vi "Standard Engine.vi"(8 "error in":errorcluster, 9 "status notifier":refnum<notifier>, 10 "rt fifo":refnum<k33>, 11 "Engine Data":T1={"Main Tag Data"={"Double"=[], "Single"=[], "I64"=[], "I32"=[], "I16"=[], "I8"=[], "U64"=[], "U32"=[], "U16"=[], "U8"=[], "Boolean"=[], "String"=[], "Array of Double"=[], "Array of Single"=[], "Array of I64"=[], "Array of I32"=[], "Array of I16"=[], "Array of I8"=[], "Array of U64"=[], "Array of U32"=[], "Array of U16"=[], "Array of U8"=[], "Array of Boolean"=[], "Array of String"=[]}, "Module Info"={"Tag Bus Modules"=[], "Input Method Indices"=[], "Process Method Indices"=[], "Output Method Indices"=[], "Input Transfer Specifications"=[], "Parameter Transfer Specifications"=[], "Result Transfer Specifications"=[], "Output Transfer Specifications"=[], "Module Errors"=[], "UID"=""}, "Safe State?"=FALSE, "engine timing source"=refnum, "Processor"=-2, "Priority"=1, "dT"=0}) -> (0 "error out":errorcluster)   [LabVIEW 2014, in "synchronous engine runtime.lvclass"]
uses:
  synchronous engine runtime.lvclass
  Engine Data.ctl
  <vilib>/NI/Module Timing Source/timing source/TBM timing source.lvclass
  <vilib>/NI/Tag Bus/table/data table.ctl
  Module Execution Info.ctl
  <vilib>/NI/Tag Bus Module Framework/runtime/TBM module execution interface.lvclass
  Data Table with Transfer Spec.ctl
  <vilib>/NI/Tag Bus/table/transfer specification.ctl
  <vilib>/NI/Tag Bus/tag/Data Type.ctl
  Commands.ctl
  notifier.ctl
  Engine Runtime/Execution States.ctl
  Engine Runtime/Engine Runtime Interface.lvclass
  <vilib>/Platform/TimedLoop/XDataNode/XDataNode.xnode
  <vilib>/Platform/TimedLoop/XDataNode/nitl_modes.ctl
  <vilib>/Platform/TimedLoop/XDataNode/XDNodeRunTimeDep.lvlib
  <vilib>/Platform/TimedLoop/XDataNode/wakeup.ctl
  <vilib>/Platform/TimedLoop/XDataNode/timing_clust.ctl
  <vilib>/NI/Tag Bus/table/data table.lvlib
  <vilib>/NI/Tag Bus/tag/tag descriptor.lvclass
panel:
  out "iterations":i32
  in  "Network Address":string="10.1.128.117"
  in  "send trace?":bool
  out "loop period (ms)":u32
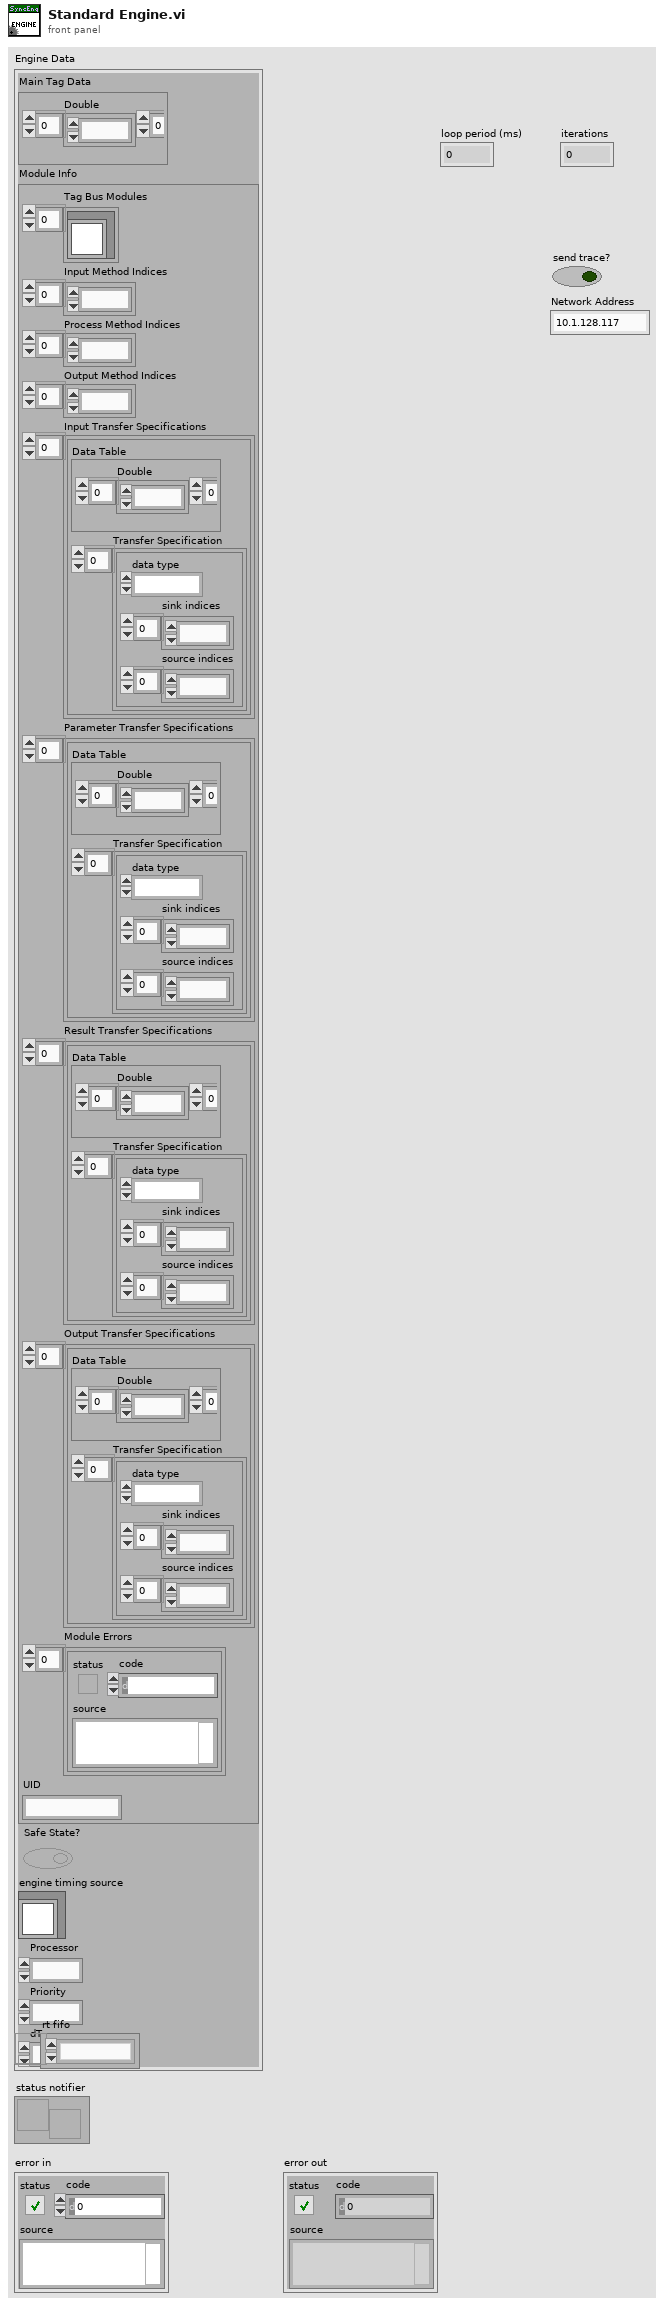
[diagram p1: front panel]
types:
  T1 = typedef "synchronous engine runtime.lvclass/Engine Data.ctl" = cluster{"Main Tag Data":T2, "Module Info":T3, "Safe State?":bool, "engine timing source":refnum<class "TBM timing source.lvclass">, "Processor":i32, "Priority":i32, "dT":u32}
  T2 = typedef "tag bus.lvlib/data table.lvlib/data table.ctl" = cluster{"Double":dbl[], "Single":sgl[], "I64":i64[], "I32":i32[], "I16":i16[], "I8":i8[], "U64":u64[], "U32":u32[], "U16":u16[], "U8":u8[], "Boolean":bool[], "String":string[], "Array of Double":cluster{"DBL Array":dbl[]}[], "Array of Single":cluster{"SGL Array":sgl[]}[], "Array of I64":cluster{"I64 Array":i64[]}[], "Array of I32":cluster{"I32 Array":i32[]}[], "Array of I16":cluster{"I16 Array":i16[]}[], "Array of I8":cluster{"I8 Array":i8[]}[], "Array of U64":cluster{"U64 Array":u64[]}[], "Array of U32":cluster{"U32 Array":u32[]}[], "Array of U16":cluster{"U16 Array":u16[]}[], "Array of U8":cluster{"U8 Array":u8[]}[], "Array of Boolean":cluster{"Boolean Array":bool[]}[], "Array of String":cluster{"String Array":string[]}[]}
  T3 = typedef "synchronous engine runtime.lvclass/Module Execution Info.ctl" = cluster{"Tag Bus Modules":refnum<class "TBM module execution interface.lvclass">[], "Input Method Indices":i32[], "Process Method Indices":i32[], "Output Method Indices":i32[], "Input Transfer Specifications":T4[], "Parameter Transfer Specifications":T4[], "Result Transfer Specifications":T4[], "Output Transfer Specifications":T4[], "Module Errors":errorcluster[], "UID":string}
  T4 = typedef "synchronous engine runtime.lvclass/Data Table with Transfer Spec.ctl" = cluster{"Data Table":T2, "Transfer Specification":T5[]}
  T5 = typedef "tag bus.lvlib/data table.lvlib/transfer specification.ctl" = cluster{"data type":T6, "sink indices":i32[], "source indices":i32[]}
  T6 = typedef "tag bus.lvlib/tag descriptor.lvclass/Data Type.ctl" = enum16{"Double", "Single", "I64", "I32", "I16", "I8", "U64", "U32", "U16", "U8", "Boolean", "String", "Array of Double", "Array of Single", "Array of I64", "Array of I32", "Array of I16", "Array of I8", "Array of U64", "Array of U32", "Array of U16", "Array of U8", "Array of Boolean", "Array of String"}
  T7 = typedef "Engine Runtime Interface.lvclass/Execution States.ctl" = enum16{"Init", "Pre-Operational", "Safe-Operational", "Operational", "Stopped"}
  T8 = typedef "synchronous engine runtime.lvclass/notifier.ctl" = cluster{"Engine State":T7, "error constant":errorcluster}
  T9 = typedef "synchronous engine runtime.lvclass/Commands.ctl" = enum16{"Start", "Pause", "Safe State", "Normal", "Stop", "Shutdown"}
  T10 = typedef "XDNodeRunTimeDep.lvlib/timing_clust.ctl" = cluster{"Expected End [f-1]":u64, "Actual End [f-1]":u64, "Finished Late? [f-1]":bool, "Expected End [i-1]":u64, "Actual End [i-1]":u64, "Finished Late? [i-1]":bool, "Expected Start [i]":u64, "Actual Start [i]":u64, "Expected Start [f]":u64, "Actual Start [f]":u64, "Source Name":string, "Structure Name":string, "Period":i64, "Deadline":i64, "Offset":i64, "Start":i64, "Priority":i32, "Timeout":i32, "Mode":T11, "Wakeup Reason":T12, "Error":errorcluster, "Source Type":string, "Secondary Source Type":string, "Global End Time":u64, "Global Start Time":u64, "Frame Duration":u64, "Iteration Duration":u64, "Assigned CPU":i32, "I/O Scan Engine Mode":u32}
  T11 = typedef "XDNodeRunTimeDep.lvlib/nitl_modes.ctl" = enum32{"No Change", "Process missed periods, maintain original phase", "Discard missed periods, maintain original phase", "Process missed periods, ignore original phase", "Discard missed periods, ignore original phase"}
  T12 = typedef "XDNodeRunTimeDep.lvlib/wakeup.ctl" = enum32{"Normal", "Aborted", "Asynchronous wakeup", "Timing source error", "Timed loop error", "Timeout"}
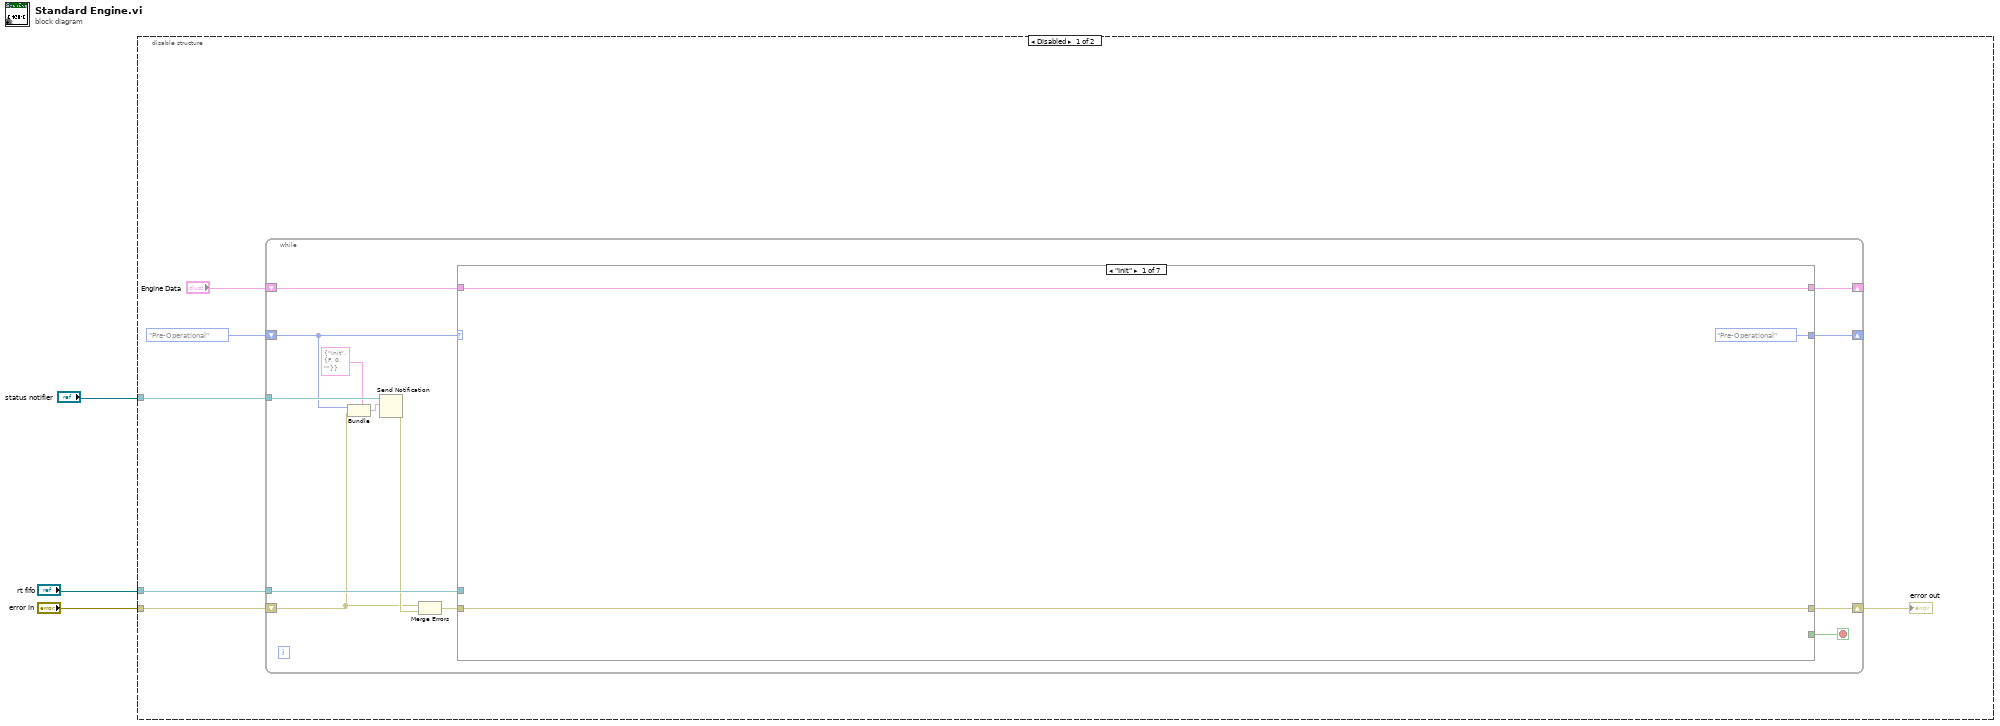
[diagram p0: block diagram]
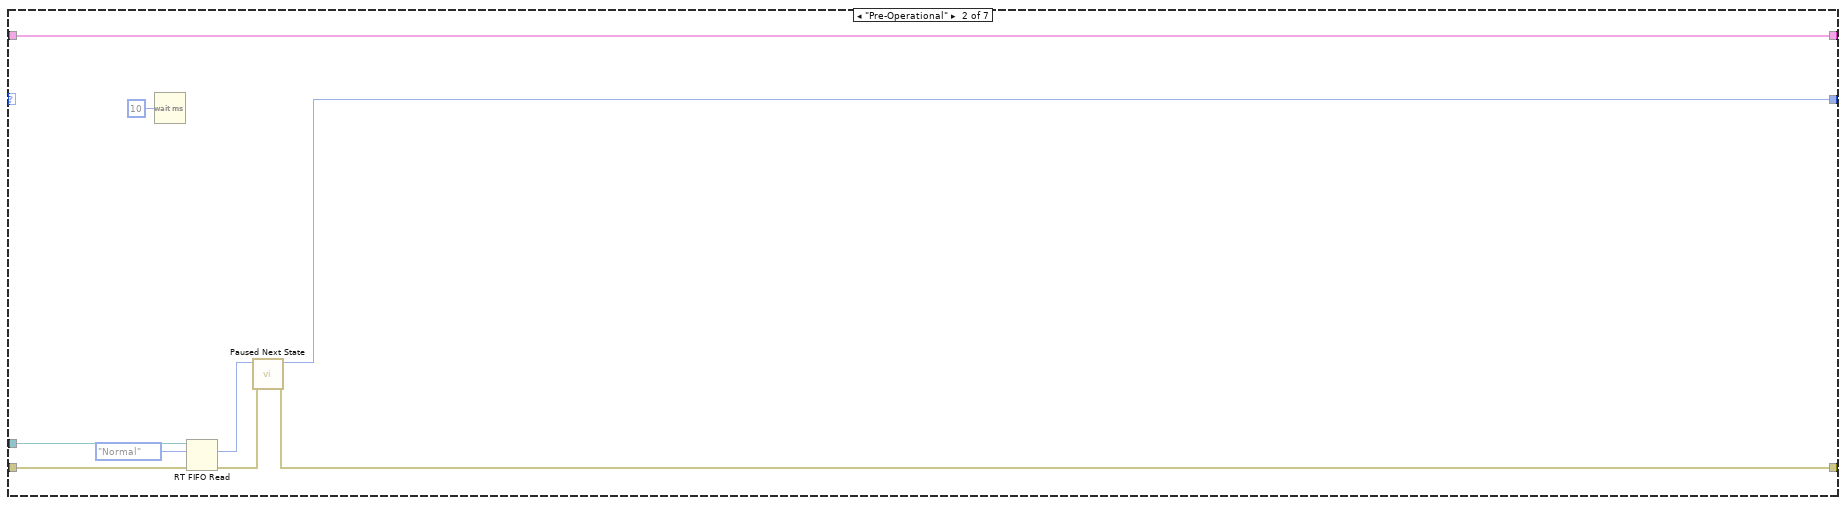
[diagram p2: hidden frame]
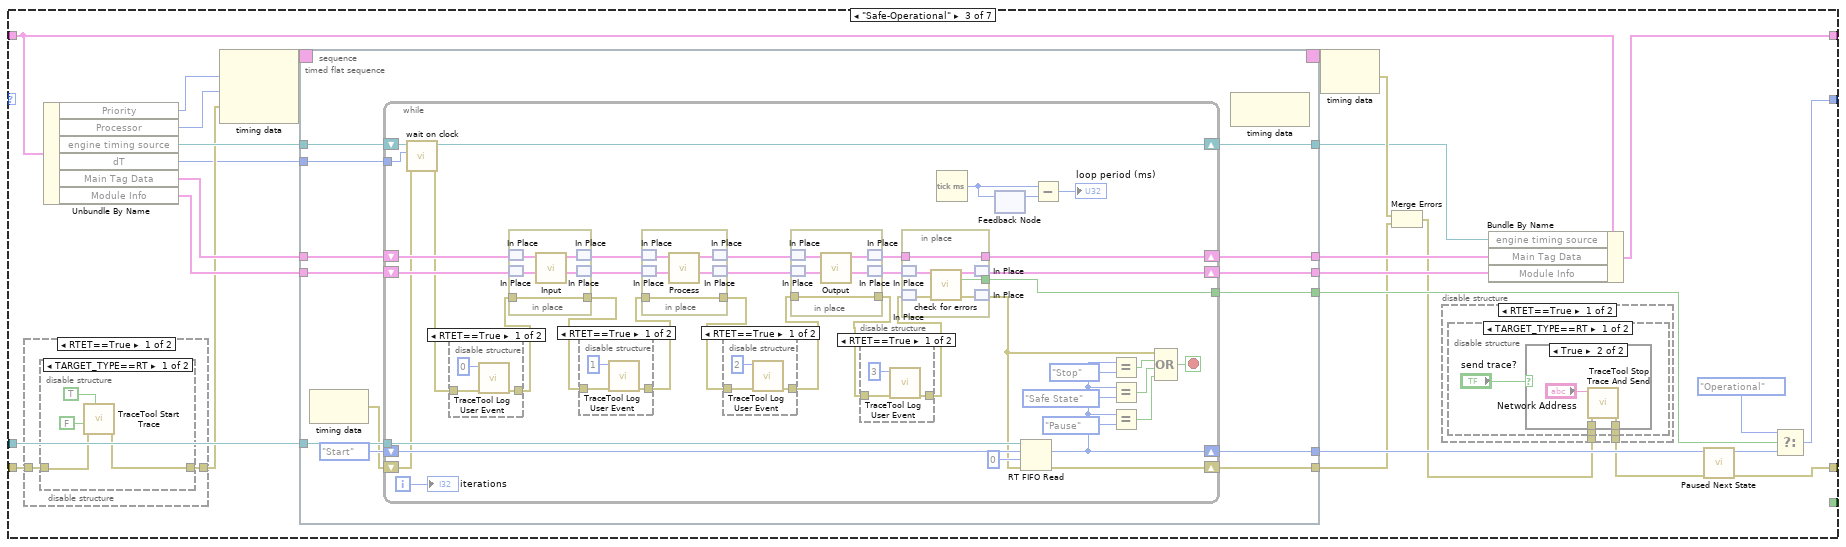
[diagram p3: hidden frame]
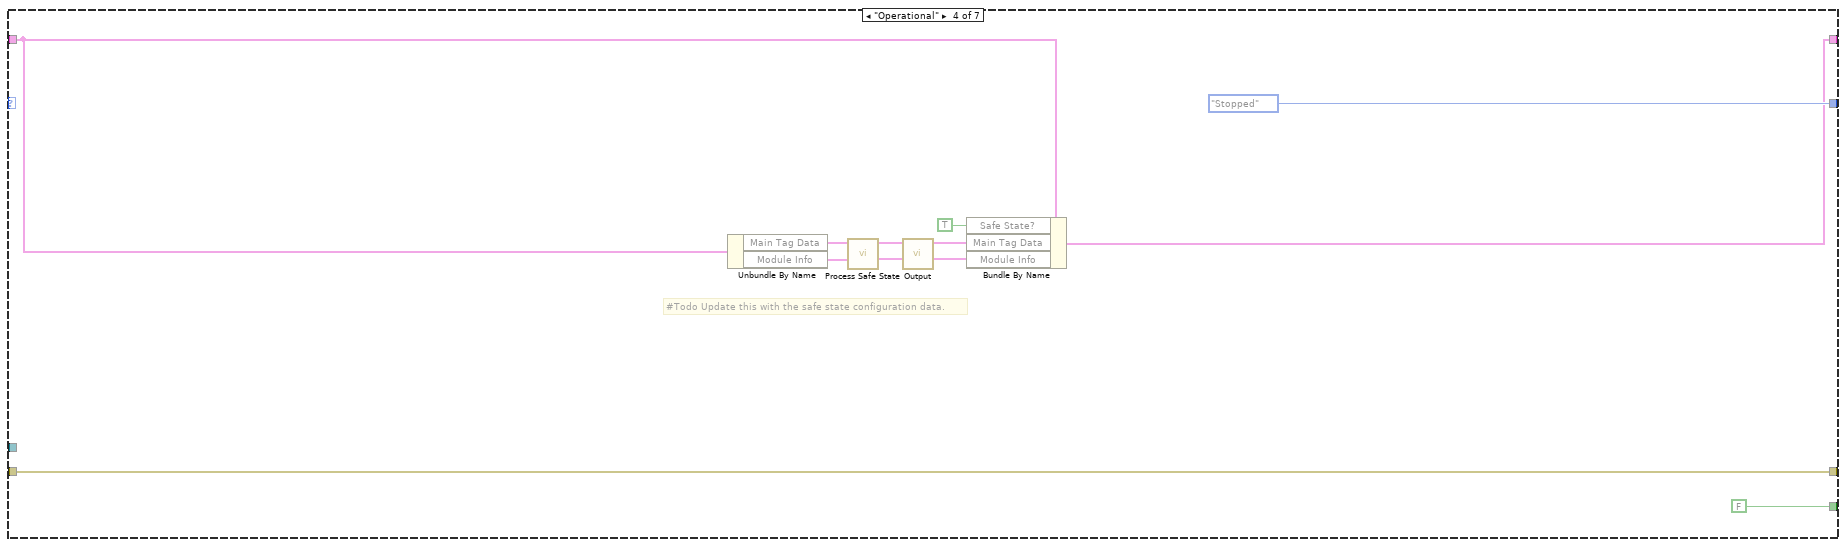
[diagram p13: hidden frame]
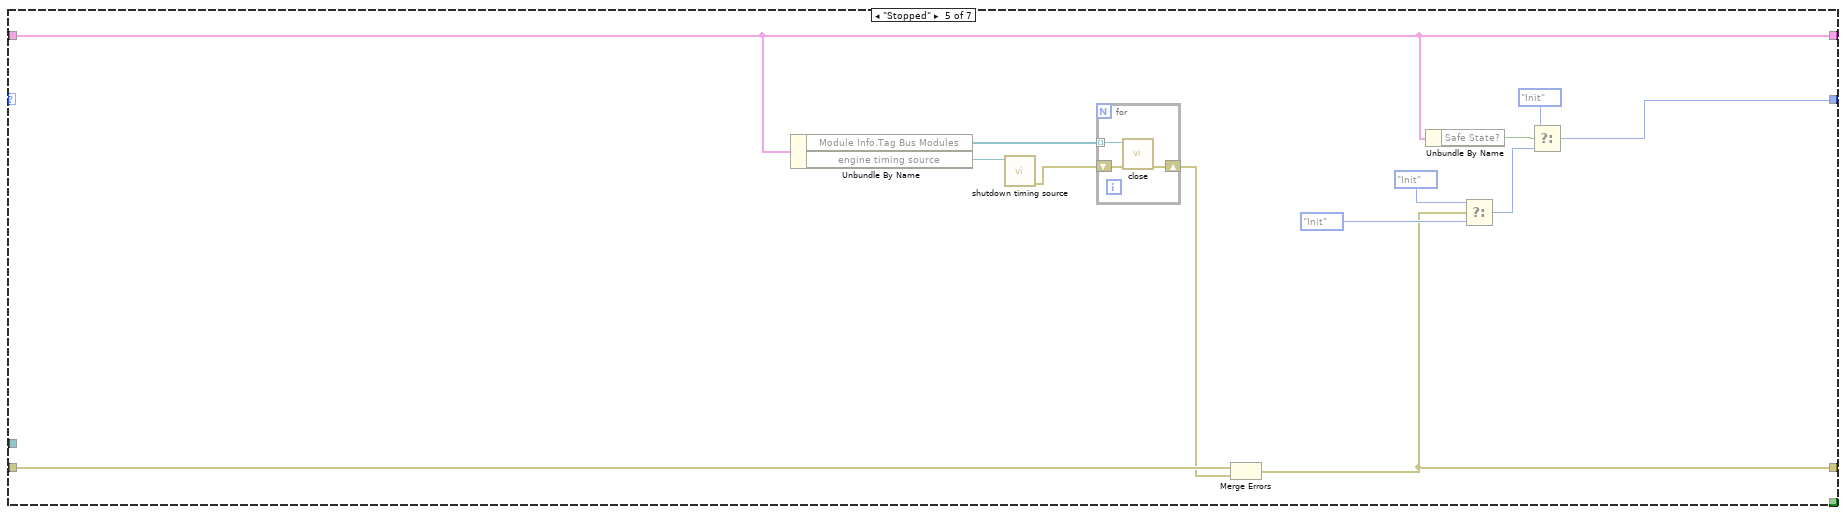
[diagram p14: hidden frame]
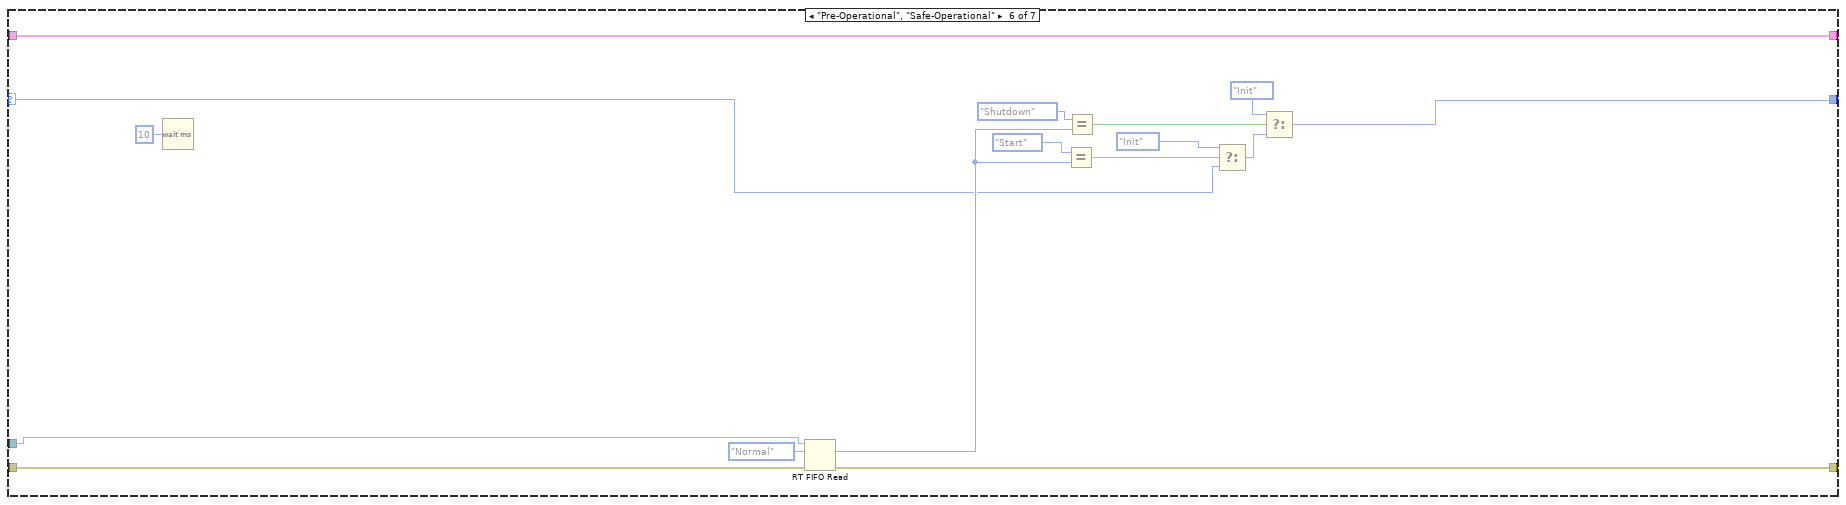
[diagram p15: hidden frame]
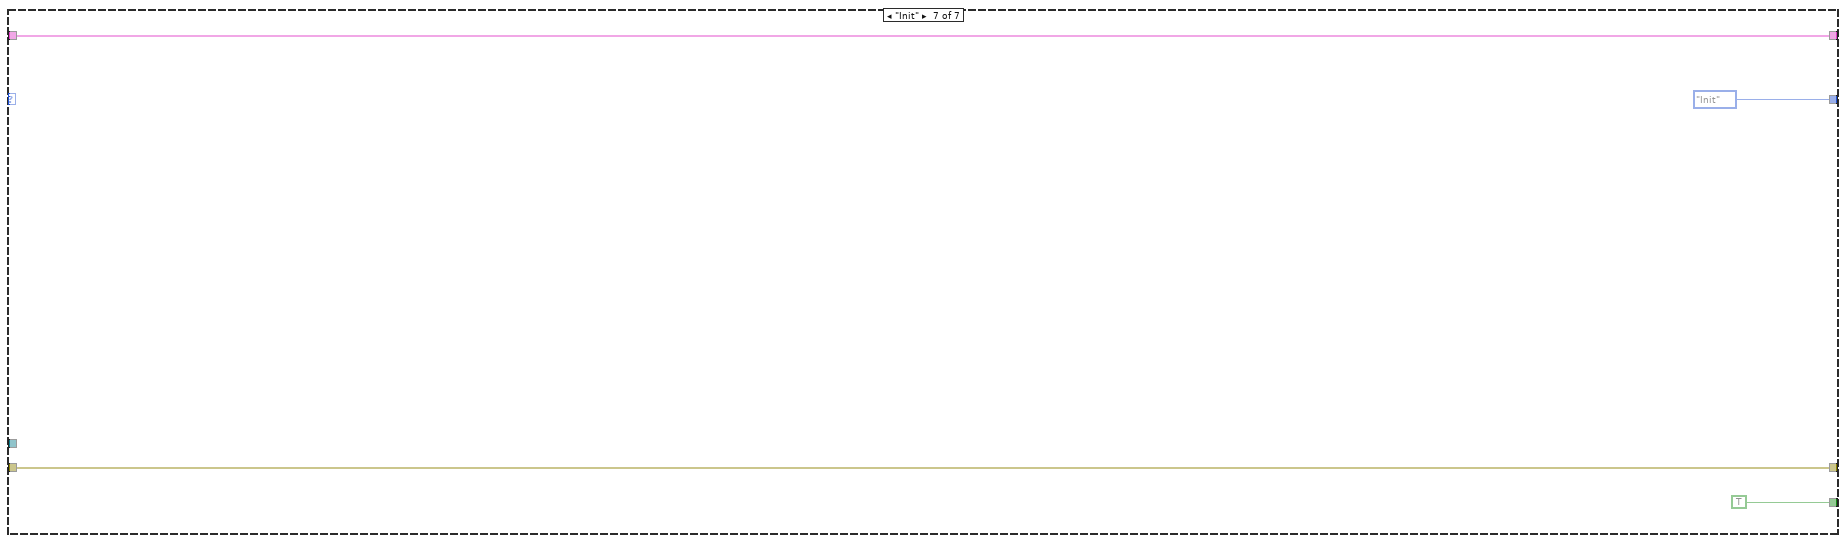
[diagram p16: hidden frame]
diagram:
  n1 = disable-structure shown="Disabled" {
    disable-tunnel: "error in" -> [w7 _]
    disable-tunnel: "status notifier" -> [w6 _]
    disable-tunnel: "rt fifo" -> [w4 _]
    frame Disabled {
      n2 = while {
        shift-right: [w19] -> _
        shift-left: Execution_States."Pre-Operational" ("States") -> [w13]
        shift-right: [w20] -> _
        shift-left: "Engine Data" -> [w22]
        shift-right: [w21] -> w8
        shift-left: w7 -> [w10]
        tunnel: w4 -> [w18]
        tunnel: w6 -> [w16]
        stop <- w17 stop-if-true
        n3 = Bundle(cluster=T8 {"Engine State"=enum."Init", "error constant"={"status"=FALSE, "code"=0, "source"=""}} ("notification"), "Engine State"=w13, "error constant"=w10) -> (w12:T8)
        n4 = Send Notification(notification=w12, notifier=w16) -> (error out=w15:errorcluster)  [unwired: 1 in, 1 out]
        n5 = Merge Errors(w10, w15) -> (w11:errorcluster)
        n6 = case shown="\"Init\"" w13 {
          selector: w13 -> [_ _ _ _ _ w220 _]
          tunnel: w22 -> [w25 w34 w36 w194 w204 w219 w236]
          tunnel: w11 -> [w24 w33 w48 w202 w208 w222 w238]
          tunnel: [w24 w27 w53 w202 w206 w229 w238] -> w21
          tunnel: [w25 w34 w37 w193 w204 w219 w236] -> w20
          tunnel: [Execution_States."Pre-Operational" ("States") w31 w49 Execution_States."Stopped" ("States") w210 w231 Execution_States."Init" ("States")] -> w19
          tunnel: w18 -> [_ w26 w60 _ _ w221 _]
          tunnel: [_ _ _ FALSE _ _ TRUE] -> w17
          frame "Init" {
          }
          frame "Pre-Operational" {
            n7 = Wait (ms)(milliseconds to wait=u32 10) -> ()  [unwired: 1 out]
            n8 = RT FIFO Read(0:w26, 1:Commands."Normal" ("Commands"), 3:w33) -> (9:w30:T9, 11:w29:errorcluster)  [unwired: 1 in, 3 out]
            n9 = call "Paused Next State.vi"("error in"=w29, "Command"=w30) -> ("error out"=w27:errorcluster, "State"=w31:T7)  [unwired: 8 in]
          }
          frame "Safe-Operational" {
            n10 = disable-structure shown="RTET==True" {
              disable-tunnel: w48 -> [w184 w190]
              disable-tunnel: [w183 w190] -> w43
              frame condition #0 {
                n11 = disable-structure shown="TARGET_TYPE==RT" {
                  disable-tunnel: w184 -> [w185 w189]
                  disable-tunnel: [w186 w189] -> w183
                  frame condition #0 {
                    n12 = call <vilib>:"TraceTool Start Trace.vi"("Detailed Tracing? (F)"=TRUE, "error in (no error)"=w185, "VI Tracing? (T)"=FALSE) -> ("error out"=w186:errorcluster)  [unwired: 7 in, 1 out]
                  }
                  frame condition #1 (active) {
                  }
                }
              }
              frame condition #1 (active) {
              }
            }
            n13 = Unbundle By Name(w36) -> ("Priority"=w38:i32, "Processor"=w39:i32, "engine timing source"=w44:refnum<class "TBM timing source.lvclass">, "dT"=w35:u32, "Main Tag Data"=w59:T2, "Module Info"=w58:T3)
            n14 = node-c288(w38, w39, w43) -> (w41:T10)
            n15 = timed-sequence {
              timing: w41 -> [_]
              timing-out: [_] -> w40
              tunnel: w60 -> [w71]
              tunnel: w59 -> [w70]
              tunnel: w58 -> [w69]
              tunnel: [w68] -> w57
              tunnel: [w67] -> w56
              tunnel: [w66] -> w55
              tunnel: [w65] -> w51
              tunnel: [w64] -> w47
              tunnel: w44 -> [w62]
              tunnel: [w63] -> w42
              tunnel: w35 -> [w61]
              n16 = timed-flat-sequence {
                tunnel: w71 -> [w84]
                tunnel: w70 -> [w82]
                tunnel: w69 -> [w81]
                tunnel: [w80] -> w68
                tunnel: [w79] -> w67
                tunnel: [w78] -> w66
                tunnel: [w77] -> w65
                tunnel: [w75] -> w64
                tunnel: [w74] -> w63
                tunnel: w62 -> [w73]
                tunnel: w61 -> [w72]
                n17 = node-c288() -> (w76:errorcluster)  [unwired: 1 in]
                n18 = while {
                  tunnel: w84 -> [w107]
                  shift-right: [w115] -> w78
                  shift-left: Commands."Start" ("Commands") -> [w127]
                  shift-right: [w104] -> w80
                  shift-left: w82 -> [w125]
                  shift-right: [w119] -> w79
                  shift-left: w81 -> [w124]
                  tunnel: [w102] -> w77
                  shift-right: [w106] -> w75
                  shift-left: w76 -> [w91]
                  shift-right: [w89] -> w74
                  shift-left: w73 -> [w92]
                  tunnel: w72 -> [w88]
                  i -> [w101]
                  stop <- w108 stop-if-true
                  n19 = call-dynamic "wait on clock.vi"("error in"=w91, "dt"=w88, "timing source in"=w92) -> ("error out"=w90:errorcluster, "timing source out"=w89:refnum<class "TBM timing source.lvclass">)  [unwired: 6 in, 1 out]
                  n20 = disable-structure shown="RTET==True" {
                    disable-tunnel: w90 -> [w142 w143]
                    disable-tunnel: [w141 w143] -> w99
                    frame condition #0 {
                      n21 = call <vilib>:"TraceTool Log User Event.vi"("error in (no error)"=w142, "Event ID (0-255)"=u32 0) -> ("error out"=w141:errorcluster)  [unwired: 9 in]
                    }
                    frame condition #1 (active) {
                    }
                  }
                  n22 = in-place {
                    in-place-border: w99 -> [w164]
                    in-place-border: [w164] -> w98
                    n23 = in-place-match #1(w125) -> (w163:T2)
                    n24 = in-place-match #2(w124) -> (w160:T3)
                    n25 = call "Input.vi"("Module Info In"=w160, "Engine Tags In"=w163) -> ("Module Info Out"=w161:T3, "Engine Tags Out"=w162:T2)  [unwired: 8 in]
                    n26 = in-place-match #1(w162) -> (w123:T2)
                    n27 = in-place-match #2(w161) -> (w122:T3)
                  }
                  n28 = disable-structure shown="RTET==True" {
                    disable-tunnel: w98 -> [w138 w139]
                    disable-tunnel: [w137 w139] -> w97
                    frame condition #0 {
                      n29 = call <vilib>:"TraceTool Log User Event.vi"("error in (no error)"=w138, "Event ID (0-255)"=u32 1) -> ("error out"=w137:errorcluster)  [unwired: 9 in]
                    }
                    frame condition #1 (active) {
                    }
                  }
                  n30 = in-place {
                    in-place-border: w97 -> [w159]
                    in-place-border: [w159] -> w96
                    n31 = in-place-match #3(w123) -> (w158:T2)
                    n32 = in-place-match #4(w122) -> (w155:T3)
                    n33 = call "Process.vi"("Module Info In"=w155, "Engine Tags In"=w158) -> ("Module Info Out"=w156:T3, "Engine Tags Out"=w157:T2)  [unwired: 8 in]
                    n34 = in-place-match #3(w157) -> (w100:T2)
                    n35 = in-place-match #4(w156) -> (w121:T3)
                  }
                  n36 = disable-structure shown="RTET==True" {
                    disable-tunnel: w96 -> [w134 w135]
                    disable-tunnel: [w133 w135] -> w95
                    frame condition #0 {
                      n37 = call <vilib>:"TraceTool Log User Event.vi"("error in (no error)"=w134, "Event ID (0-255)"=u32 2) -> ("error out"=w133:errorcluster)  [unwired: 9 in]
                    }
                    frame condition #1 (active) {
                    }
                  }
                  n38 = in-place {
                    in-place-border: w95 -> [w154]
                    in-place-border: [w154] -> w94
                    n39 = in-place-match #5(w100) -> (w153:T2)
                    n40 = in-place-match #6(w121) -> (w152:T3)
                    n41 = call "Output.vi"("Module Info In"=w152, "Engine Tags In"=w153) -> ("Module Info Out"=w151:T3, "Engine Tags Out"=w150:T2)  [unwired: 8 in]
                    n42 = in-place-match #5(w150) -> (w103:T2)
                    n43 = in-place-match #6(w151) -> (w120:T3)
                  }
                  n44 = disable-structure shown="RTET==True" {
                    disable-tunnel: w94 -> [w130 w131]
                    disable-tunnel: [w129 w131] -> w93
                    frame condition #0 {
                      n45 = call <vilib>:"TraceTool Log User Event.vi"("error in (no error)"=w130, "Event ID (0-255)"=u32 3) -> ("error out"=w129:errorcluster)  [unwired: 9 in]
                    }
                    frame condition #1 (active) {
                    }
                  }
                  n46 = in-place {
                    in-place-border: [w149] -> w104
                    in-place-border: w103 -> [w149]
                    in-place-border: [w144] -> w102
                    n47 = in-place-match #7(w120) -> (w147:T3)
                    n48 = in-place-match #8(w93) -> (w145:errorcluster)
                    n49 = call "check for errors.vi"("error in"=w145, "Module Info in"=w147) -> ("error out"=w146:errorcluster, "safe state"=w144:bool, "Module Info out"=w148:T3)  [unwired: 7 in]
                    n50 = in-place-match #7(w148) -> (w119:T3)
                    n51 = in-place-match #8(w146) -> (w105:errorcluster)
                  }
                  n52 = Tick Count (ms)() -> (millisecond timer value=w118:u32)
                  n53 = feedback-in #9(w118) -> ()
                  n54 = feedback #9() -> (w117:u32)  [unwired: 1 in]
                  n55 = RT FIFO Read(0:w107, 1:w127, 2:0 ("timeout in ms (0)"), 3:w105) -> (9:w115:T9, 11:w106:errorcluster)  [unwired: 3 out]
                  n56 = Subtract(x=w118, y=w117) -> (x-y=→"loop period (ms)":u32)
                  n57 = Equal?(x=w115, y=Commands."Stop") -> (x = y?=w111:bool)
                  n58 = Equal?(x=w115, y=Commands."Safe State") -> (x = y?=w110:bool)
                  n59 = Equal?(x=w115, y=Commands."Pause") -> (x = y?=w109:bool)
                  n60 = Compound Arithmetic op=OR(w105, w111, w110, w109) -> (w108:bool)
                  "iterations" <- w101
                }
                n61 = node-c288() -> ()  [unwired: 1 in, 1 out]
              }
            }
            n62 = node-c288(w40) -> (w45:errorcluster)
            n63 = Merge Errors(w45, w47) -> (w46:errorcluster)
            n64 = disable-structure shown="RTET==True" {
              disable-tunnel: [w173 w182] -> w54
              disable-tunnel: w46 -> [w172 w182]
              frame condition #0 {
                n65 = disable-structure shown="TARGET_TYPE==RT" {
                  disable-tunnel: [w176 w181] -> w173
                  disable-tunnel: w172 -> [w175 w181]
                  frame condition #0 {
                    n66 = case shown="True" "send trace?" {
                      tunnel: [w177 w180] -> w176
                      tunnel: w175 -> [w177 w179]
                      frame False {
                      }
                      frame True {
                        n67 = call <vilib>:"TraceTool Stop Trace And Send.vi"("error in (no error)"=w179, "Trace Host Network Address"="Network Address") -> ("error out"=w180:errorcluster)  [unwired: 9 in]
                      }
                    }
                  }
                  frame condition #1 (active) {
                  }
                }
              }
              frame condition #1 (active) {
              }
            }
            n68 = Bundle By Name(cluster=w36, "engine timing source"=w42, "Main Tag Data"=w57, "Module Info"=w56) -> (w37:T1)
            n69 = call "Paused Next State.vi"("error in"=w54, "Command"=w55) -> ("error out"=w53:errorcluster, "State"=w52:T7)  [unwired: 8 in]
            n70 = Select(t=Execution_States."Operational", s=w51, f=w52) -> (s? t:f=w49:T7)
          }
          frame "Operational" {
            # "#Todo Update this with the safe state configuration data."
            n71 = Unbundle By Name(w194) -> ("Main Tag Data"=w192:T2, "Module Info"=w191:T3)
            n72 = call "Process Safe State.vi"("Module Info In"=w191, "Engine Tags In"=w192) -> ("Module Info Out"=w197:T3, "Engine Tags Out"=w198:T2)  [unwired: 8 in]
            n73 = call "Output.vi"("Module Info In"=w197, "Engine Tags In"=w198) -> ("Module Info Out"=w195:T3, "Engine Tags Out"=w196:T2)  [unwired: 8 in]
            n74 = Bundle By Name(cluster=w194, "Safe State?"=TRUE, "Main Tag Data"=w196, "Module Info"=w195) -> (w193:T1)
          }
          frame "Stopped" {
            n75 = Unbundle By Name(w204) -> ("Module Info.Tag Bus Modules"=w215:refnum<class "TBM module execution interface.lvclass">[], "engine timing source"=w205:refnum<class "TBM timing source.lvclass">)
            n76 = call-dynamic "shutdown timing source.vi"("timing source in"=w205) -> ("error out"=w209:errorcluster)  [unwired: 9 in, 1 out]
            n77 = for {
              tunnel: w215 -> [w216] mode=indexing
              shift-right: [w217] -> w207
              shift-left: w209 -> [w218]
              n78 = call-dynamic "close.vi"("error in"=w218, "module in"=w216) -> ("error out"=w217:errorcluster)  [unwired: 9 in]
            }
            n79 = Merge Errors(w208, w207) -> (w206:errorcluster)
            n80 = Unbundle By Name(w204) -> ("Safe State?"=w203:bool)
            n81 = Select(t=Execution_States."Init" ("States"), s=w206, f=Execution_States."Init" ("States")) -> (s? t:f=w211:T7)
            n82 = Select(t=Execution_States."Init" ("States"), s=w203, f=w211) -> (s? t:f=w210:T7)
          }
          frame "Pre-Operational", "Safe-Operational" {
            n83 = Wait (ms)(milliseconds to wait=u32 10) -> ()  [unwired: 1 out]
            n84 = RT FIFO Read(0:w221, 1:Commands."Normal" ("Commands"), 3:w222) -> (9:w234:T9, 11:w229:errorcluster)  [unwired: 1 in, 3 out]
            n85 = Equal?(x=Commands."Start" ("Commands"), y=w234) -> (x = y?=w233:bool)
            n86 = Equal?(x=Commands."Shutdown" ("Commands"), y=w234) -> (x = y?=w228:bool)
            n87 = Select(t=Execution_States."Init" ("States"), s=w233, f=w220) -> (s? t:f=w232:T7)
            n88 = Select(t=Execution_States."Init" ("States"), s=w228, f=w232) -> (s? t:f=w231:T7)
          }
          frame "Init" {
          }
        }
      }
      "error out" <- w8
    }
    frame Enabled {
    }
  }
